vi "Search VI.vi"(9 "DependencyPaths":path[](array[path]), 11 "Expected VIs":path[](array[path])) -> (1 "VIs Relative Path":path[](array[path]), 2 "VIs":path[](array[path]), 3 "vi references":refnum<vi>[](array[refnum]))   [LabVIEW 2019, in "Language Selection.lvlib"]
doc: "Converts VI's path from relative to absolute.\n- - -\nCopyright (c) 2026, Merecs Engineering GmbH"
uses:
  Language Selection.lvlib
panel:
  # "Connector Pane"
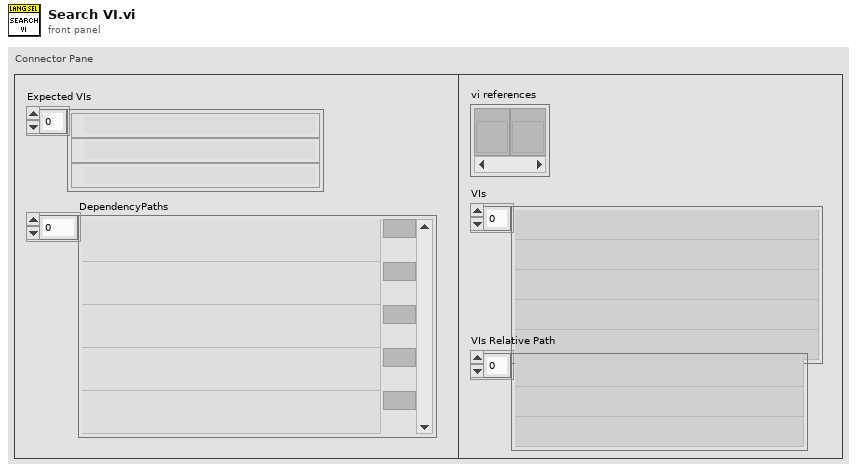
[diagram p1: front panel]
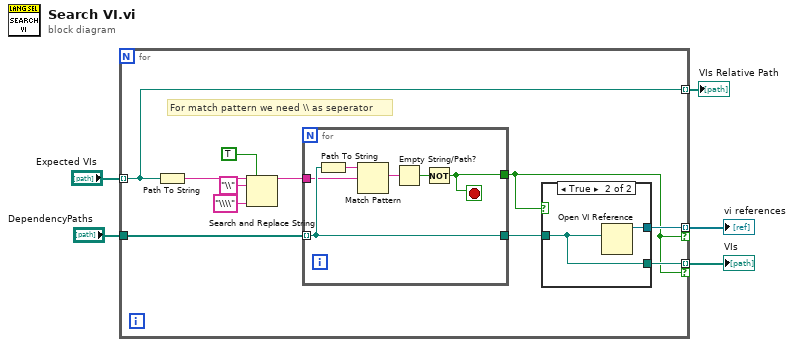
[diagram p0: block diagram]
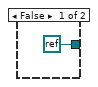
[diagram p2: hidden frame]
diagram:
  n1 = for {
    tunnel: "DependencyPaths" -> [w16]
    tunnel: "Expected VIs" -> [w6] mode=indexing
    tunnel: [w15] -> w5 mode=indexing if=w7
    tunnel: [w8] -> w2 mode=indexing if=w7
    tunnel: [w6] -> w1 mode=indexing
    # "For match pattern we need \\\\ as seperator"
    n2 = Path To String(path=w6) -> (string=w10:string)
    n3 = Search and Replace String(replace all?=TRUE ("replace all? (F)"), input string=w10, search string="\\", replace string="\\\\" ("replace string (\"\")")) -> (result string=w11:string)  [unwired: 4 in, 3 out]
    n4 = for {
      tunnel: w16 -> [w19] mode=indexing
      tunnel: w11 -> [w17]
      tunnel: [w19] -> w14
      tunnel: [w20] -> w7
      stop <- w20 stop-if-true
      n5 = Path To String(path=w19) -> (string=w18:string)
      n6 = Match Pattern(string=w18, regular expression=w17) -> (match substring=w22:string)  [unwired: 1 in, 3 out]
      n7 = Empty String/Path?(string/path=w22) -> (empty?=w21:bool)
      n8 = Not(x=w21) -> (.not. x?=w20:bool)
    }
    n9 = case shown="True" w7 {
      tunnel: w14 -> [_ w24]
      tunnel: [refnum<k0> refnum w25] -> w15
      tunnel: [_ w24] -> w8
      frame False {
      }
      frame True {
        n10 = Open VI Reference(vi path=w24) -> (vi reference=w25:refnum<vi>)  [unwired: 5 in, 1 out]
      }
    }
  }
  "vi references" <- w5
  "VIs" <- w2
  "VIs Relative Path" <- w1
